vi "cvTypeToImageType.vi"(10 "error in":errorcluster, 11 "cvType":T2) -> (2 "error out":errorcluster, 3 "Image Type":T1)   [LabVIEW 2020, in "OpenLvVision_OpenCv.lvlib"]
uses:
  OpenLvVision_OpenCv.lvlib
  <vilib>/OpenLvVision/OpenLvVision_Image/Management/TypeDef/OLV ImageType.ctl
  <vilib>/OpenLvVision/OpenLvVision_Image/Management/OLV Management.lvlib
  <vilib>/ErrorRing/Error Ring.xnode
  <vilib>/Utility/error.llb/Error Cluster From Error Code.vi
  TypeDef/cvType.ctl
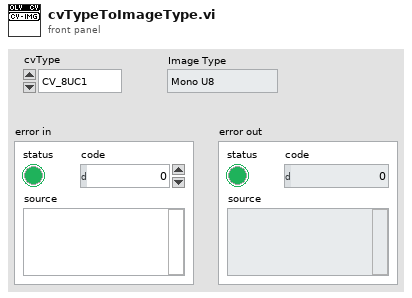
[diagram p1: front panel]
types:
  T1 = typedef "OLV OpenLvVision_Image.lvlib/OLV Management.lvlib/OLV ImageType.ctl" = enum16{"Mono U8", "Mono U16", "Mono I16", "Mono SGL", "Color U32", "Color U64", "Complex CSG"}
  T2 = typedef "OpenLvVision_OpenCv.lvlib/cvType.ctl" = enum32{"CV_8UC1", "CV_8SC1", "CV_16UC1", "CV_16SC1", "CV_32SC1", "CV_32FC1", "CV_64FC1", "CV_16FC1", "CV_8UC2", "CV_8SC2", "CV_16UC2", "CV_16SC2", "CV_32SC2", "CV_32FC2", "CV_64FC2", "CV_16FC2", "CV_8UC3", "CV_8SC3", "CV_16UC3", "CV_16SC3", "CV_32SC3", "CV_32FC3", "CV_64FC3", "CV_16FC3", "CV_8UC4", "CV_8SC4", "CV_16UC4", "CV_16SC4", "CV_32SC4", "CV_32FC4", "CV_64FC4", "CV_16FC4"}
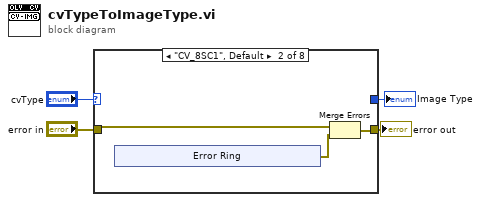
[diagram p0: block diagram]
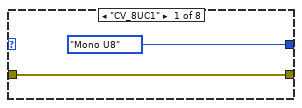
[diagram p2: hidden frame]
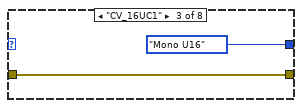
[diagram p3: hidden frame]
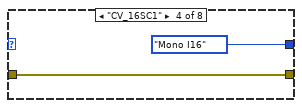
[diagram p4: hidden frame]
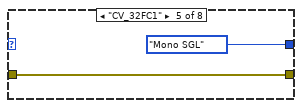
[diagram p5: hidden frame]
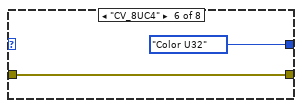
[diagram p6: hidden frame]
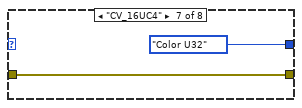
[diagram p7: hidden frame]
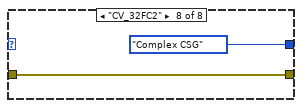
[diagram p8: hidden frame]
diagram:
  n1 = case shown="\"CV_8SC1\", Default" "cvType" {
    tunnel: "error in" -> [w6 w8 w15 w17 w19 w21 w23 w26]
    tunnel: [w6 w9 w15 w17 w19 w21 w23 w26] -> w2
    tunnel: [OLV_ImageType."Mono U8" ("Image Type") _ OLV_ImageType."Mono U16" ("Image Type") OLV_ImageType."Mono I16" ("Image Type") OLV_ImageType."Mono SGL" ("Image Type") OLV_ImageType."Color U32" ("Image Type") OLV_ImageType."Color U32" ("Image Type") OLV_ImageType."Complex CSG" ("Image Type")] -> w1
    frame "CV_8UC1" {
    }
    frame "CV_8SC1", Default {
      n2 = xnode "Error Ring"() -> ("error out"=w7:errorcluster)
      n3 = Merge Errors(w8, w7) -> (w9:errorcluster)
    }
    frame "CV_16UC1" {
    }
    frame "CV_16SC1" {
    }
    frame "CV_32FC1" {
    }
    frame "CV_8UC4" {
    }
    frame "CV_16UC4" {
    }
    frame "CV_32FC2" {
    }
  }
  "Image Type" <- w1
  "error out" <- w2
